vi "Acquisition.vi"(7 "Name(\"\" to use uuid)":string="Acquisition") -> ()   [LabVIEW 2017, in "Acquisition.lvlib"]
uses:
  Acquisition.lvlib
  _support/Hardware Configuration.ctl
  _support/Signal Type.ctl
  bc6f9ce3-7135-4df3-9fce-67397201bd09.vi
  f3e3012a-dc83-45d7-82c5-490bef76f43f.vi
  e2413101-be31-4c43-921b-7e7496268bc5.vi
  07cbb487-6694-43fd-ac53-f2be3466fcff.vi
  fecb174d-6823-407c-a974-ffebb4610b14.vi
  0bf643a1-791c-4b4c-b91f-da80b9c7e2fb.vi
  041ba748-83ae-40d3-86c4-8e2f4b565384.vi
  <userlib>/_NEVSTOP/Communicable State Machine(CSM)/AdvanceAPI/CSM - Revert Arguments-Safe String.vi
  <userlib>/_NEVSTOP/Communicable State Machine(CSM)/_Shared/Trim Single-line Text.vi
  <userlib>/_NEVSTOP/Communicable State Machine(CSM)/AdvanceAPI/CSM - Make String Arguments Safe.vi
  <userlib>/_NEVSTOP/Communicable State Machine(CSM)/AdvanceAPI/CSM - Break Down Multiple States String.vi
  <userlib>/_NEVSTOP/Communicable State Machine(CSM)/AdvanceAPI/CSM - Compact Multiple States.vi
  f3e3012a-dc83-45d7-82c5-490bef76f43f.vi/99de0c97-112a-4c86-9094-c187659127e1.vi
  <userlib>/_NEVSTOP/Communicable State Machine(CSM)/Utility/Build Error Cluster.vi
  0bf643a1-791c-4b4c-b91f-da80b9c7e2fb.vi/99de0c97-112a-4c86-9094-c187659127e1.vi
  <userlib>/_NEVSTOP/Communicable State Machine(CSM)/AdvanceAPI/CSM - Keywords.vi
  <vilib>/Utility/Data Type/Get Type Information.vi
  <userlib>/_NEVSTOP/Communicable State Machine(CSM)/addons/API-String-Arugments-Support/_Support/Data To SingleElementsArray_csm.vi
  <userlib>/_NEVSTOP/Communicable State Machine(CSM)/addons/API-String-Arugments-Support/_Support/Data To API String Arguments.vi
  <userlib>/_NEVSTOP/Communicable State Machine(CSM)/addons/INI-Static-Variable-Support/_Support/Parse Used Session and Name.vi
  <userlib>/_NEVSTOP/Communicable State Machine(CSM)/addons/INI-Static-Variable-Support/_Support/INI-FGV(lvlibp).vi
  <userlib>/_NEVSTOP/Communicable State Machine(CSM)/addons/INI-Static-Variable-Support/_Support/Populate String with INI Variable.vi
  <userlib>/_NEVSTOP/Communicable State Machine(CSM)/addons/API-String-Arugments-Support/_Support/Convert API String Arguments to Data(variant).vi
  <userlib>/_NEVSTOP/Communicable State Machine(CSM)/addons/API-String-Arugments-Support/_Support/SingleElementsArray To Data_csm.vi
  <userlib>/_NEVSTOP/Communicable State Machine(CSM)/addons/API-String-Arugments-Support/_Support/Query Data as API String Arguments(variant).vi
  <userlib>/_NEVSTOP/Communicable State Machine(CSM)/addons/MassData-Parameter/_support/FGV-MassData(lvlibp).vi
  <userlib>/_NEVSTOP/Communicable State Machine(CSM)/_Polymophic/Add State(s) to Queue By BOOL(Element).vi
  <userlib>/_NEVSTOP/Communicable State Machine(CSM)/_Polymophic/CSM - Filter Duplicated Lines.vi
  <userlib>/_NEVSTOP/Communicable State Machine(CSM)/_Polymophic/CSM - Replace Marks in Messages.vi
  <userlib>/_NEVSTOP/Communicable State Machine(CSM)/Communicable State Machine.lvlib
  <userlib>/_NEVSTOP/Communicable State Machine(CSM)/addons/Loop-Support/CSM Loop Support.lvlib
  <userlib>/_NEVSTOP/Communicable State Machine(CSM)/_Shared/CSM Shared.lvlib
panel:
  in  "Signal Type":enum16{"Sine Wave", "Square with Noise"}(ring)
  in  "Cancel Button":bool
  in  "OK Button":bool
  out "Error Occurred":errorcluster
  out "State History":string
  # "Configure The Simulated Waveform Type"
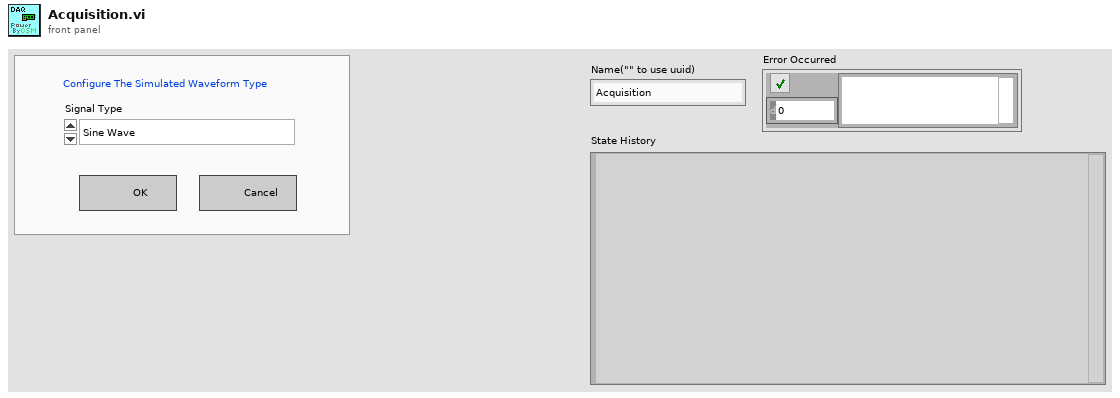
[diagram p1: front panel]
types:
  T1 = enum32{"Invalid", "Default", "Floating", "Floating/Auto-Hide", "Modal"}
  T2 = typedef "Acquisition.lvlib/Hardware Configuration.ctl" = cluster{"Resource":string, "SignalType":T3}
  T3 = typedef "Acquisition.lvlib/Signal Type.ctl" = enum16{"Sine Wave", "Square with Noise"}
  T4 = enum32{"Invalid", "Standard", "Closed", "Hidden", "Minimized", "Maximized"}
  T5 = enum32{"invalid app kind", "Development System", "Run Time System", "Student Edition", "Embedded LabVIEW", "Evaluation", "Custom"}
  T6 = typedef "Communicable State Machine.lvlib/_CSM_Response Source Message.ctl" = cluster{"‘State":string, "’Arguments":string, "’Error":errorcluster}
  T7 = cluster{"Current VI Reference":refnum<vi>, "Close Panel on Exit?":bool}
  T8 = cluster{"Core":cluster{"Current VI Reference":refnum<vi>, "Close Panel on Exit?":bool}, "Configuration":T2, "State":enum16{"Idle", "Acquiring"}, "SamplePeroid(ms)":u32}
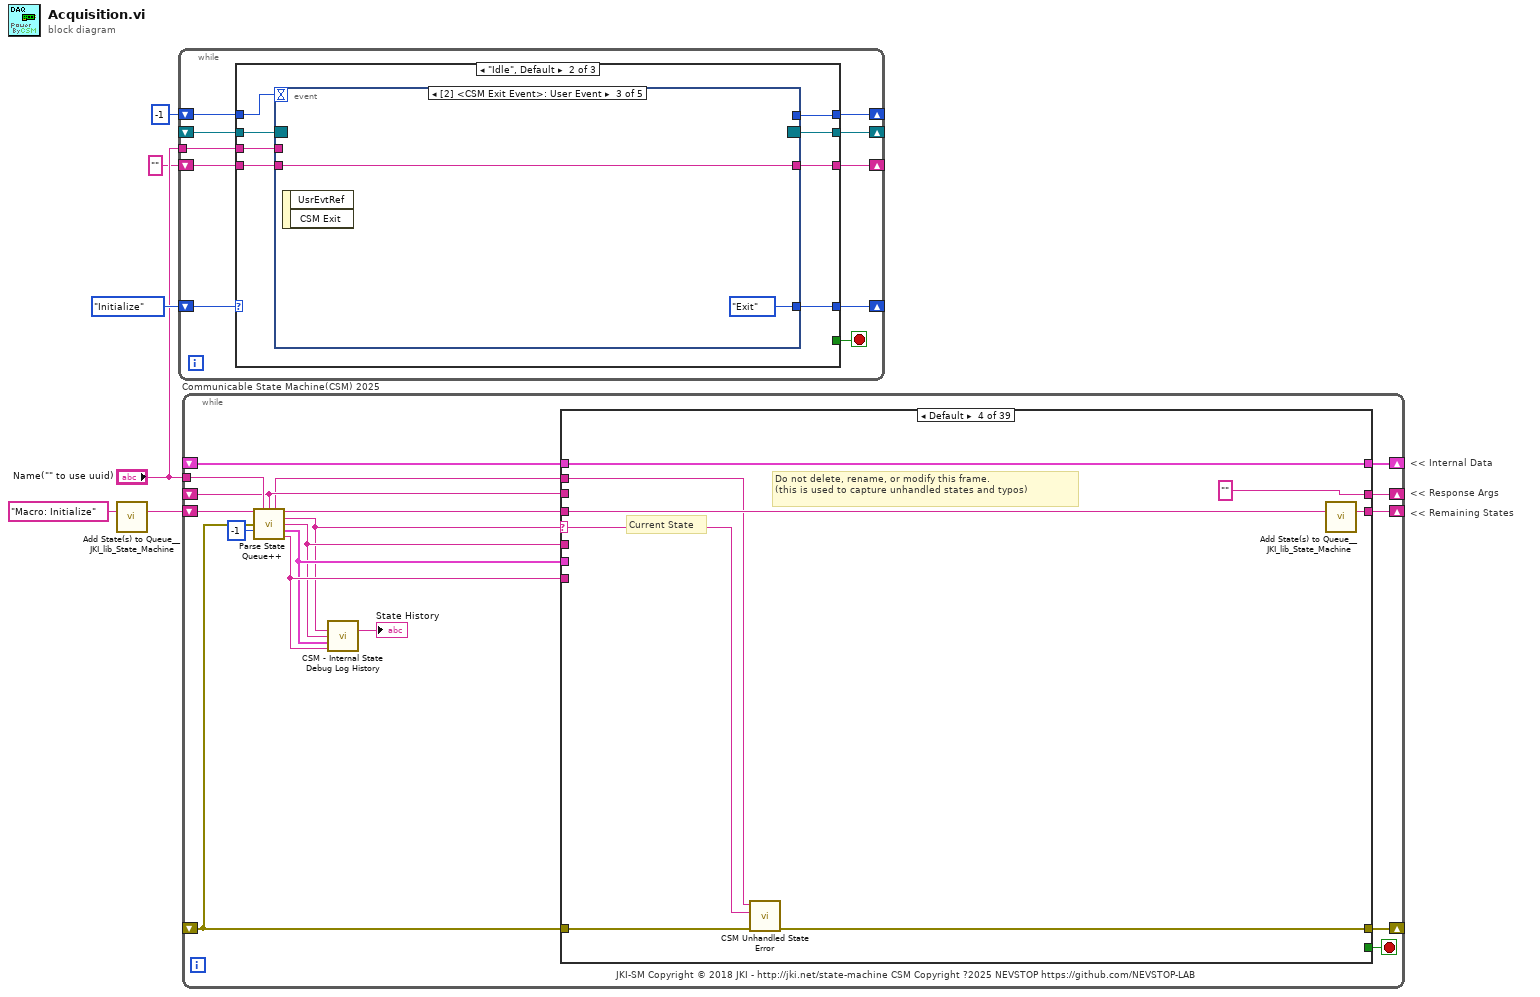
[diagram p0: block diagram]
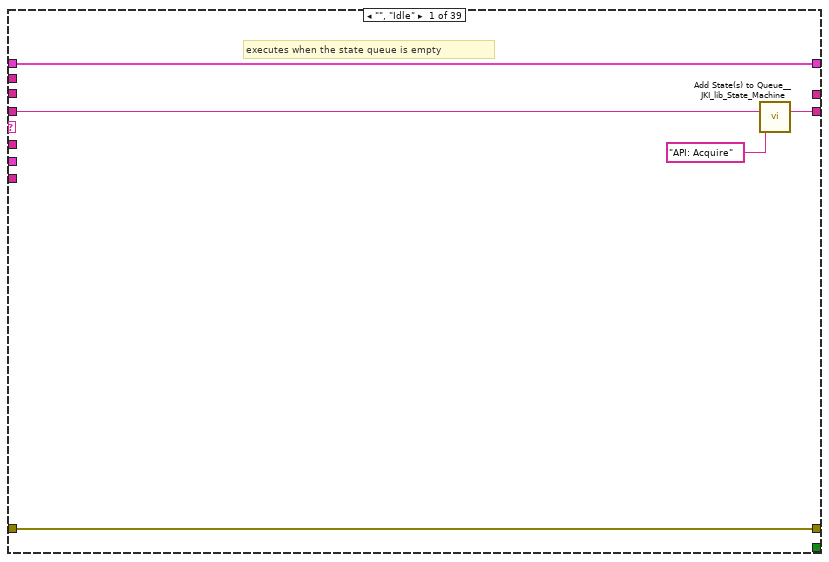
[diagram p2: hidden frame]
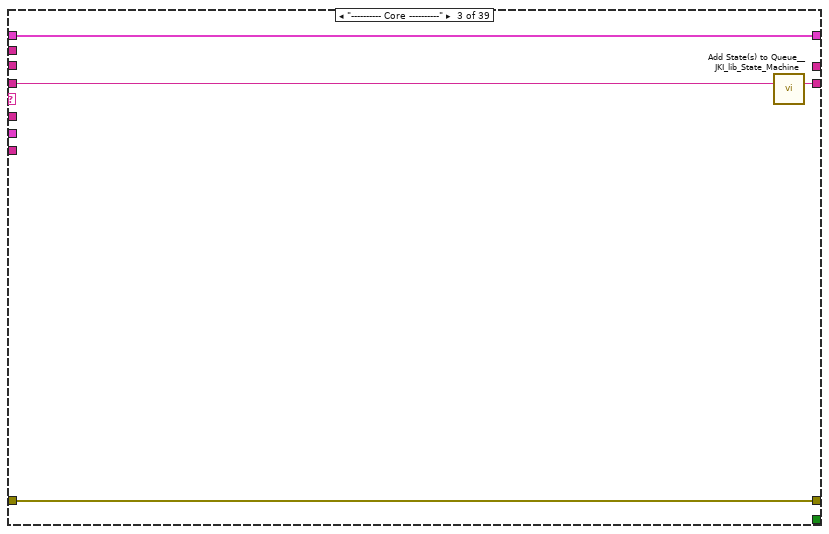
[diagram p4: hidden frame]
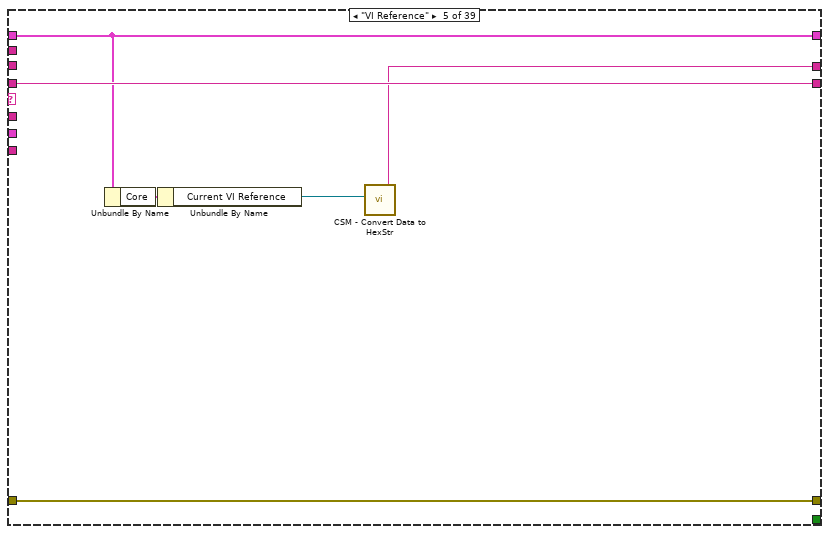
[diagram p5: hidden frame]
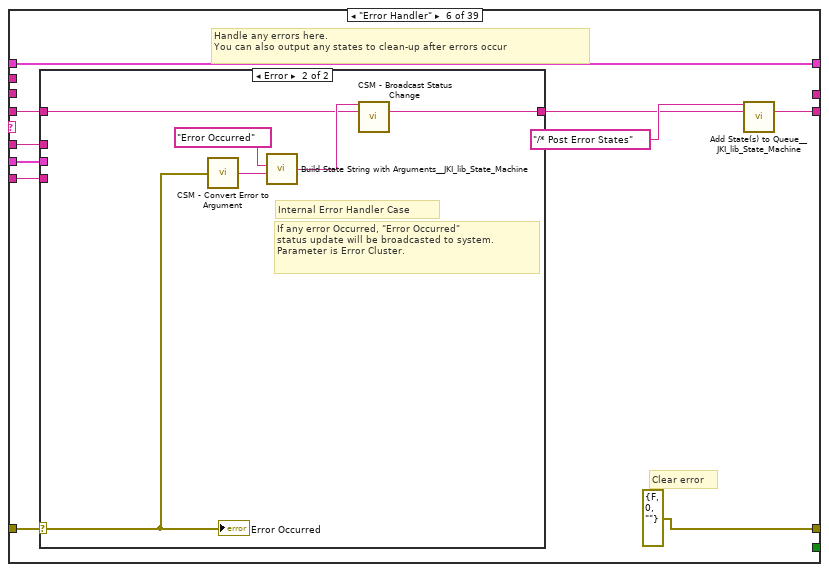
[diagram p6: hidden frame]
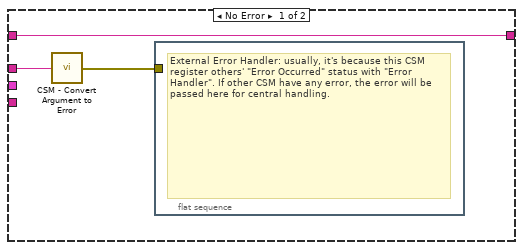
[diagram p7: hidden frame]
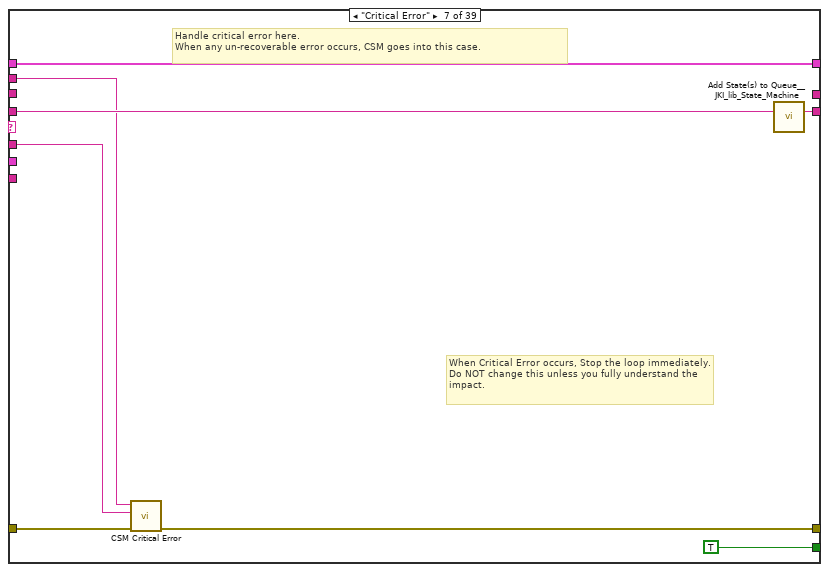
[diagram p8: hidden frame]
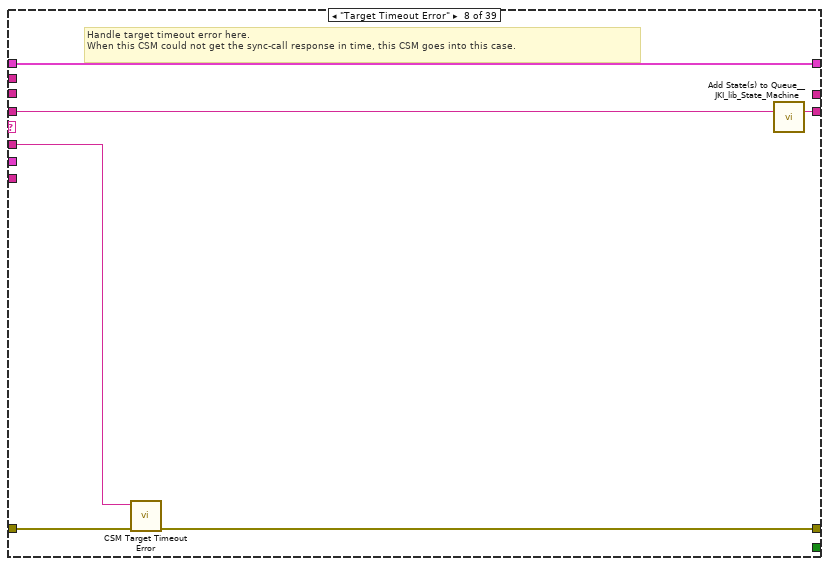
[diagram p9: hidden frame]
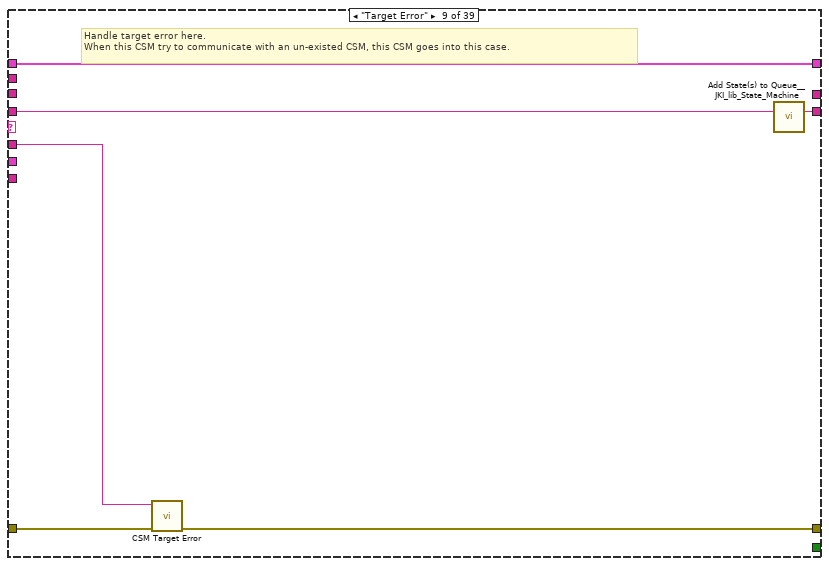
[diagram p10: hidden frame]
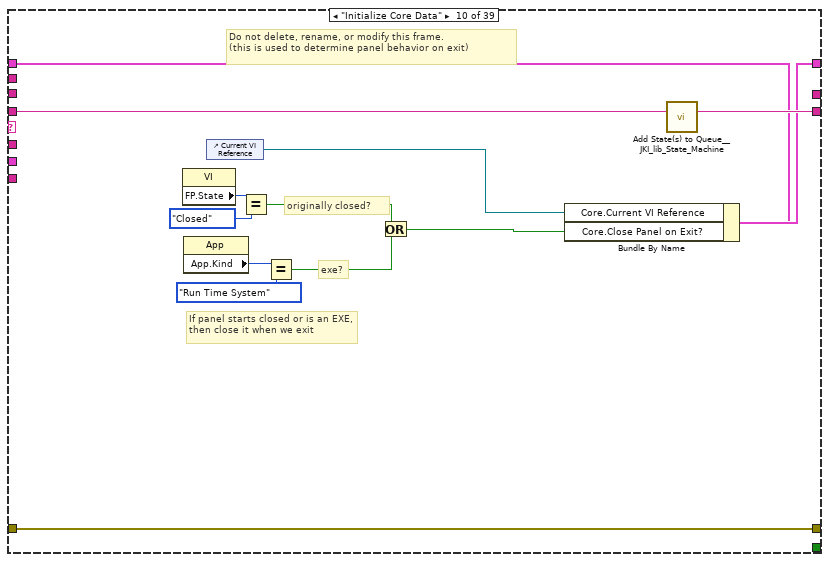
[diagram p11: hidden frame]
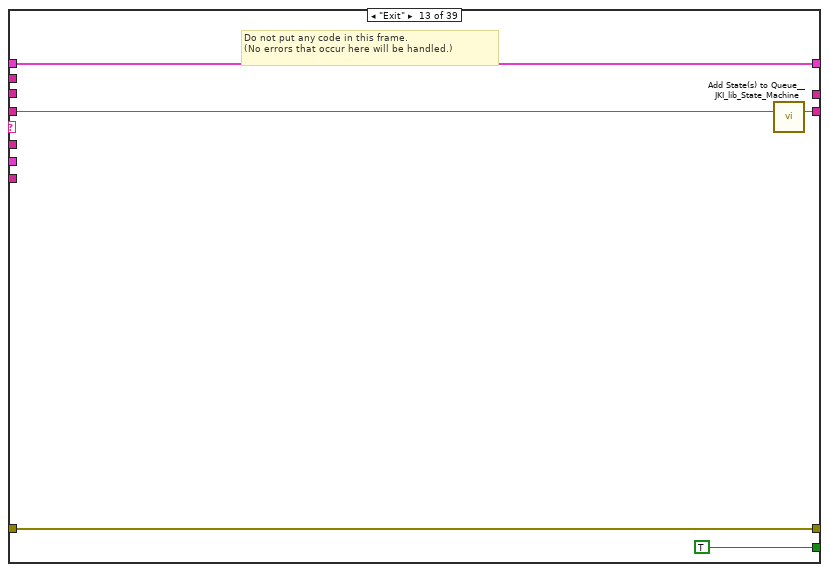
[diagram p14: hidden frame]
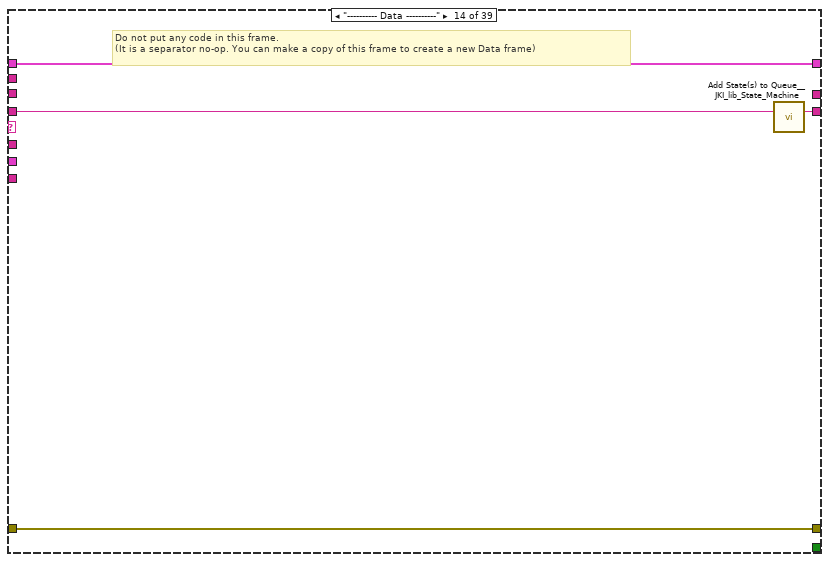
[diagram p15: hidden frame]
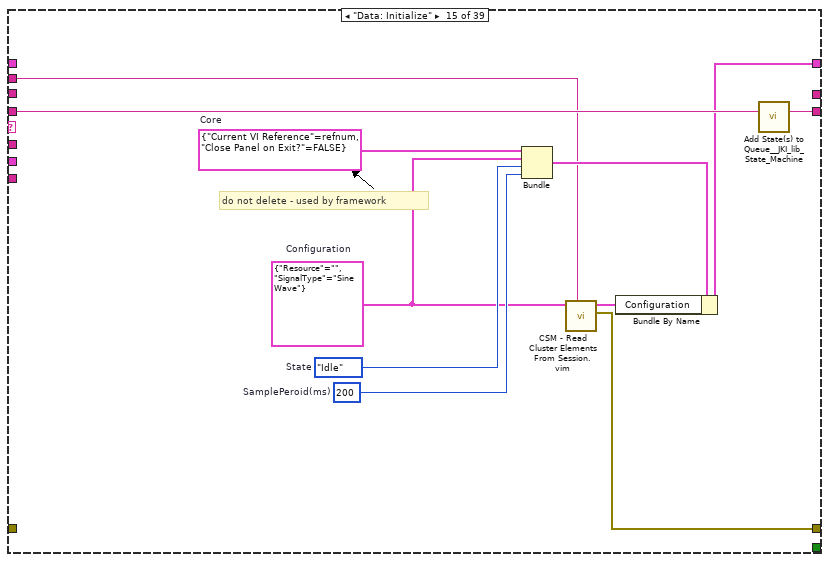
[diagram p16: hidden frame]
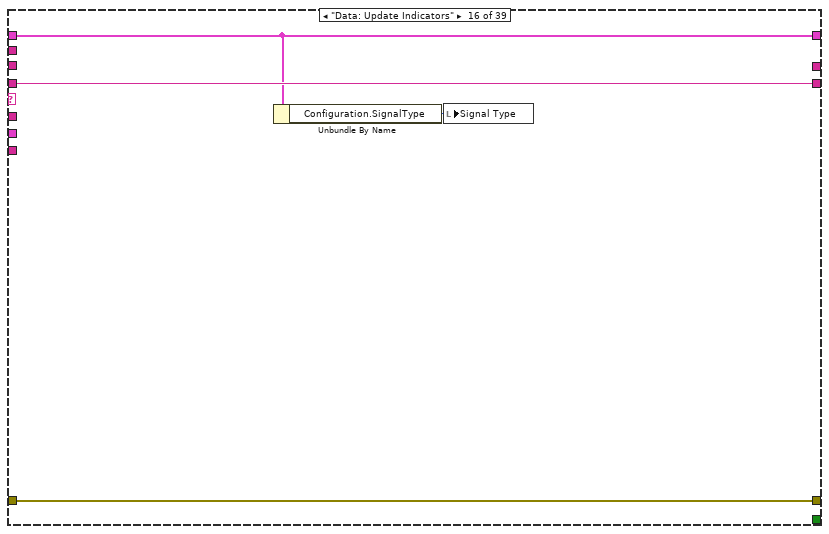
[diagram p17: hidden frame]
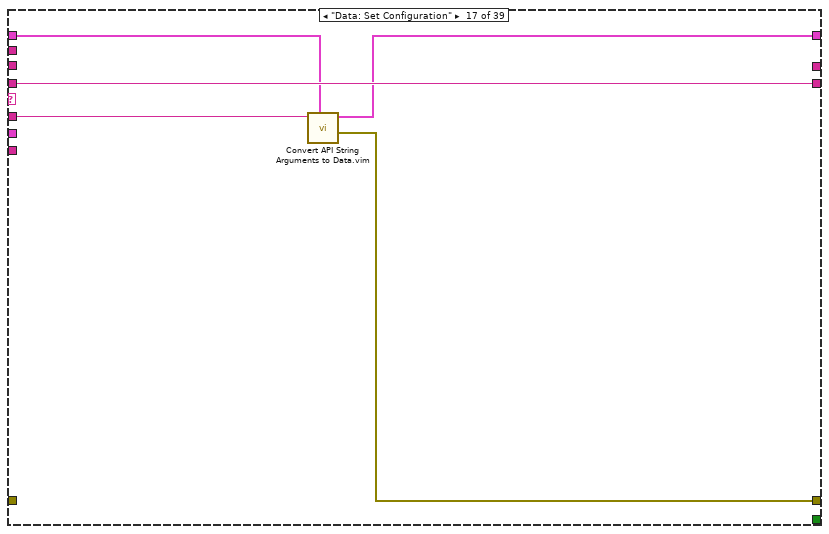
[diagram p18: hidden frame]
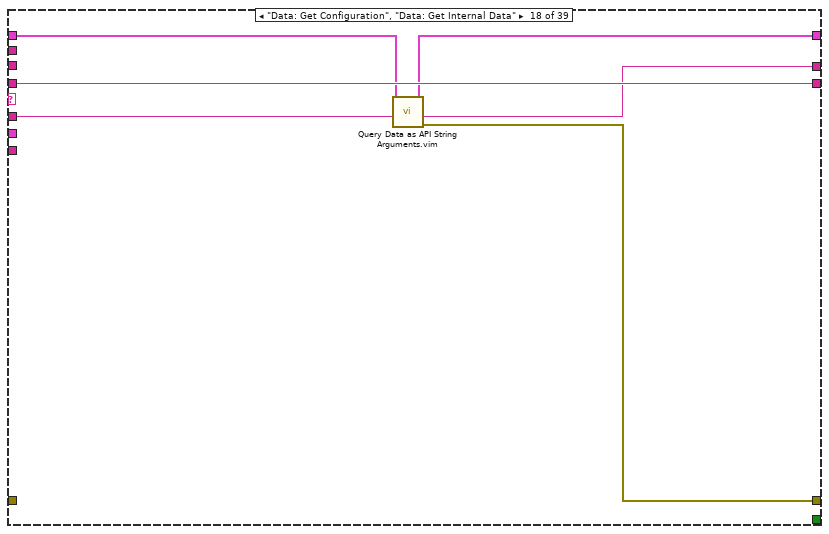
[diagram p19: hidden frame]
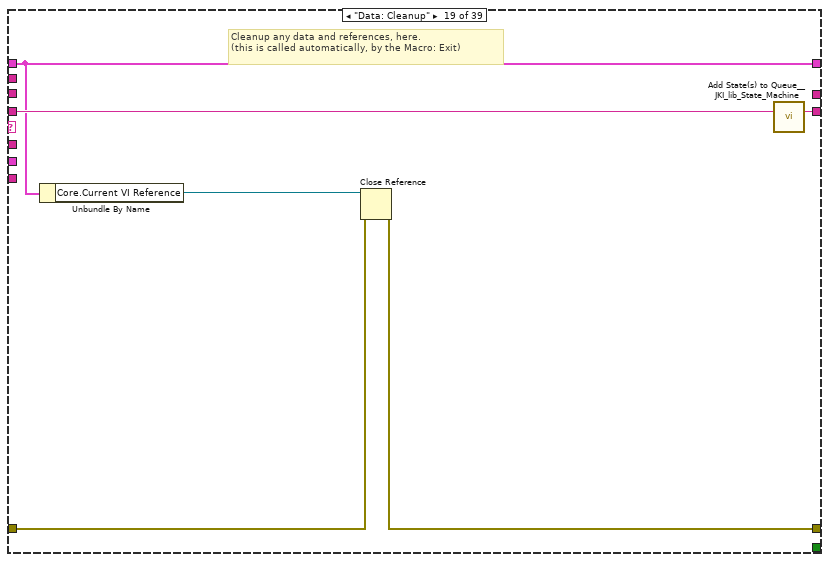
[diagram p20: hidden frame]
diagram:
  # "<< Internal Data"
  # "<< Response Args"
  # "<< Remaining States"
  n1 = call <vilib>:"Add State(s) to Queue__JKI_lib_State_Machine.vi"("State(s) in (\"\")"="Macro: Initialize") -> ("States Out"=w5:string)  [unwired: 14 in]
  n2 = while {
    shift-right: [w12] -> _
    shift-left: enum16{"Idle", "Initialize", "Exit"}."Initialize" -> [w16]
    tunnel: "Name(\"\" to use uuid)" -> [w15]
    shift-right: [w14] -> _
    shift-left: _ -> [w13]
    shift-right: [w9] -> _
    shift-left: "" -> [w10]
    shift-right: [w7] -> _
    shift-left: -1 -> [w8]
    stop <- w11 stop-if-true
    n3 = case shown="\"Idle\", Default" w16 {
      tunnel: w15 -> [w25 w29 _]
      tunnel: [w22 w34 _] -> w14
      tunnel: w13 -> [_ w33 w62]
      tunnel: [enum16{"Idle", "Initialize", "Exit"}."Idle" w32 _] -> w12
      tunnel: [_ _ TRUE] -> w11
      tunnel: w10 -> [w19 w31 w59]
      tunnel: [w19 w30 w59] -> w9
      tunnel: w8 -> [w18 w27 w58]
      tunnel: [w18 w28 w58] -> w7
      frame "Initialize" {
        n4 = call <userlib>:"CSM - Wait for Module to Be Alive.vi"("CSM Name"=w25) -> ("CSM Name (Dup)"=w20:string, "error out"=w26:errorcluster)  [unwired: 12 in, 1 out]
        n5 = call <userlib>:"CSM - Module Exit Event.vi"("Error In"=w26, "Name (\"\" to Use UUID) In"=w20) -> ("error out"=w24:errorcluster, "CSM Exit Event"=w23:refnum<user-event>)  [unwired: 7 in, 1 out]
        n6 = register-events(error in=w24, w23) -> (reference out=w22:refnum<event-registration>)  [unwired: 1 in, 1 out]
        n7 = property class="VI"("FP.Behavior"=T1."Default" ("Front Panel Window:Behavior")) -> ()  [unwired: 2 in, 2 out]
      }
      frame "Idle", Default {
        n8 = event shown="[2] <CSM Exit Event>: User Event" {
          selector: w33 -> [_ _ _ _ _]
          dyn-events: [_ _ _ _ _] -> w34
          timeout: w27 -> [_ _ _ _ _]
          tunnel: [_ _ enum16{"Idle", "Initialize", "Exit"}."Exit" _ _] -> w32
          tunnel: w31 -> [w38 w42 w44 w53 w56]
          tunnel: [w39 w41 w44 w52 w55] -> w30
          tunnel: w29 -> [w36 _ _ _ _]
          tunnel: [-1 _ _ _ _] -> w28
          event Timeout {
            n9 = event-data() -> ()  [unwired: 1 in, 3 out]
            n10 = call-poly <userlib>:"CSM - Filter JKISM String Queue.vi"("States In"=w38) -> ("States Out"=w35:string)  [unwired: 14 in]
            n11 = call <userlib>:"CSM - Forward UI Operations to CSM.vi"("Name (\"\" to Use UUID)"=w36, "State(s) In (\"\")"=w35) -> ("States Out"=w39:string)  [unwired: 8 in, 1 out]
          }
          event Panel Close? {
            n12 = event-data() -> ()  [unwired: 1 in, 2 out]
            n13 = call <vilib>:"Add State(s) to Queue__JKI_lib_State_Machine.vi"("State(s) in Front (\"\")"="Do: Hide FP and Exit When stand-alone" ("State(s) in Front (\"\")"), "State(s) in (\"\")"=w42) -> ("States Out"=w41:string)  [unwired: 13 in]
            n14 = event-data("Discard?"=TRUE) -> ()  [unwired: 1 in, 1 out]
          }
          event User Event {
            n15 = event-data() -> ()  [unwired: 1 in, 2 out]
          }
          event "OK Button": Value Change {
            n16 = event-data() -> ()  [unwired: 1 in, 1 out]
            n17 = Bundle By Name(cluster=T2 {"Resource"="", "SignalType"=enum."Sine Wave"} ("Hardware Config"), "SignalType"="Signal Type") -> (w48:T2)
            n18 = call "Convert Data To API String Arguments.vim"("Data"=w48) -> ("API String"=w47:string)  [unwired: 7 in, 1 out]
            n19 = call-poly <userlib>:"Build Message with Arguments++.vi"("States With Replace Token"="API: Update Settings >> <param>\nData: Update Indicators\nDo: Hide FP and Exit When stand-alone" ("State"), "<param>"=w47) -> ("States"=w46:string)  [unwired: 13 in]
            n20 = call <vilib>:"Add State(s) to Queue__JKI_lib_State_Machine.vi"("State(s) in (\"\")"=w53, "State(s) at Back (\"\")"=w46) -> ("States Out"=w52:string)  [unwired: 13 in]
          }
          event "Cancel Button": Value Change {
            n21 = event-data() -> ()  [unwired: 1 in, 1 out]
            n22 = call <vilib>:"Add State(s) to Queue__JKI_lib_State_Machine.vi"("State(s) in Front (\"\")"="Do: Hide FP and Exit When stand-alone" ("State(s) in Front (\"\")"), "State(s) in (\"\")"=w56) -> ("States Out"=w55:string)  [unwired: 13 in]
          }
        }
      }
      frame "Exit" {
        n23 = Unregister For Events(event registration refnum=w62) -> (error out=w61:errorcluster)  [unwired: 1 in]
        n24 = call <vilib>:"Clear Errors.vi"("error in (no error)"=w61) -> ()  [unwired: 5 in, 2 out]
        n25 = property class="VI"("FP.Behavior"=T1."Default" ("Front Panel Window:Behavior")) -> ()  [unwired: 2 in, 2 out]
      }
    }
  }
  n26 = while "Communicable State Machine(CSM) 2025" {
    shift-right: [w75] -> _
    shift-left: _ -> [w65]
    shift-right: [w78] -> _
    shift-left: _ -> [w74]
    shift-right: [w77] -> _
    shift-left: w5 -> [w79]
    tunnel: "Name(\"\" to use uuid)" -> [w72]
    shift-right: [w73] -> _
    shift-left: _ -> [w67]
    stop <- w76 stop-if-true
    # "JKI-SM Copyright © 2018 JKI - http://jki.net/state-machine CSM Copyright ?2025 NEVSTOP https://github.com/NEVSTOP-LAB"
    n27 = call <userlib>:"Parse State Queue++.vi"("State Queue"=w79, "Name (\"\" to Use UUID)"=w72, "Response Arguments"=w67, "Previous Error"=w74, "Dequeue (1 ms)"=-1 ("Dequeue Timeout(1ms)")) -> ("Name Used"=w66:string, "Remaining States"=w80:string, "Current State"=w68:string, "Arguments"=w69:string, "Additional Information"=w70:T6, "Source CSM"=w71:string)  [unwired: 5 in]
    n28 = call <userlib>:"CSM - Internal State Debug Log History.vi"("State"=w68, "Arguments (\"\")"=w69, ">> Response Source Message >>"=w70, "Source (\"\")"=w71) -> ("Debug Log"=→"State History":string)  [unwired: 11 in]
    n29 = case shown="Default" w68 {
      selector: w68 -> [_ _ _ w94 _ _ _ _ _ _ _ _ _ _ _ _ _ _ _ _ _ _ _ _ _ _ _ _ _ _ _ _ _ _ w316 _ _ _ _]
      tunnel: w80 -> [w82 w87 w92 w99 w105 w110 w132 w138 w144 w158 w160 w163 w169 w173 w184 w187 w193 w199 w205 w209 w214 w219 w221 w225 w238 w251 w262 w269 w275 w280 w285 w308 w310 w313 w320 w323 w327 w334 w401]
      tunnel: w69 -> [_ _ _ _ _ w109 w128 w135 w141 _ _ _ _ _ _ _ w191 w196 _ _ _ _ _ _ _ w247 _ _ _ _ _ _ _ _ w315 _ _ w331 _]
      tunnel: w65 -> [w84 w86 w89 w97 w104 w115 w130 w136 w142 w151 w159 w162 w167 w170 _ w185 w192 w198 w200 w206 w211 w216 w220 w228 w234 w249 w261 w267 w272 w279 w287 w305 w309 w312 w318 w324 w326 w333 w410]
      tunnel: [w85 w88 w90 w95 w106 errorcluster {"status"=FALSE, "code"=0, "source"=""} ("error out") w126 w134 w140 w155 w161 w164 w166 w171 w174 w188 w189 w194 w201 w207 w212 w217 w222 w226 w236 w243 w263 w264 w270 w281 w289 w306 w311 w314 w321 w325 w328 w330 w409] -> w78
      tunnel: w74 -> [w85 w88 w90 w100 w106 w113 w133 w139 w145 w155 w161 w164 w166 w171 _ w188 _ _ w202 w207 w212 w217 w222 w226 w236 _ w263 _ _ w281 w290 _ w311 w314 w321 w325 w328 w332 w409]
      tunnel: [w83 w87 w91 w98 w105 w111 w131 w137 w143 w157 w160 w163 w168 w172 w183 w187 w193 w199 w204 w208 w213 w218 w221 w224 w237 w251 w262 w269 w275 w280 w286 w308 w310 w313 w319 w322 w327 w334 w402] -> w77
      tunnel: [_ _ _ _ _ _ TRUE _ _ _ _ _ TRUE _ _ _ _ _ _ _ _ _ _ _ _ _ _ _ _ _ _ _ _ _ _ _ _ _ _] -> w76
      tunnel: [w84 w86 w89 w97 w104 w115 w130 w136 w142 w156 w159 w162 w167 w170 w176 w185 w190 w197 w200 w206 w211 w216 w220 w227 w234 w250 w261 w265 w271 w278 w288 w304 w309 w312 w318 w324 w326 w333 w410] -> w75
      tunnel: w71 -> [_ _ _ _ _ w108 _ _ _ _ _ _ _ _ _ _ _ _ _ _ _ _ _ _ _ _ _ _ _ _ _ _ _ _ _ _ _ _ _]
      tunnel: w70 -> [_ _ _ _ _ w107 _ _ _ _ _ _ _ _ _ _ _ _ _ _ _ _ _ _ _ _ _ _ _ _ _ _ _ _ _ _ _ _ _]
      tunnel: [_ _ _ "" w101 _ _ _ _ _ _ _ _ _ _ _ _ w195 _ _ _ _ _ _ _ _ _ _ _ _ w283 _ _ _ _ _ _ _ _] -> w73
      tunnel: w66 -> [_ _ _ w93 _ _ w127 _ _ _ _ _ _ _ w178 _ _ _ _ _ _ _ _ _ _ w242 _ _ _ _ _ _ _ _ _ _ _ _ _]
      tunnel: w67 -> [_ _ _ _ _ _ _ _ _ _ _ _ _ _ _ _ _ _ _ _ _ _ _ _ _ _ _ _ _ _ _ _ _ _ _ _ _ _ _]
      frame "", "Idle" {
        # "executes when the state queue is empty"
        n30 = call <vilib>:"Add State(s) to Queue__JKI_lib_State_Machine.vi"("State(s) in (\"\")"=w82, "State(s) at Back (\"\")"="API: Acquire" ("State(s) in Front (\"\")")) -> ("States Out"=w83:string)  [unwired: 13 in]
      }
      frame "CSM Documentation" {
        # "CSM Documentation"
        # "State Syntax:\nStateCategory: State >> Argument -@ CSMName\nStateCategory: State >> Argument -> CSMName\n\nLine Terminator: Line feed"
        # "Commenting:\nTo add a comment use \"//\" or \"#\" and all text to the right will be ignored\nCommenting Example:\nUI: Initialize // This initializes the UI\n// Another comment line"
        # "Example:\nUI: Help >> About -@Main\nUI: Help >> About ->Main\n\nWhere \"UI\" is the state category\nWhere \"Help\" is the state\nWhere \"About\" is the argument\nWhere \"Main\" is the Name of CSM,which actually run the \"UI: Help >> About\"\n\n    \"-@\" stands for sync state. Current CSM will wait until the state is finished. \n            - if \"Main\" named CSM does not exist, \"Target Error\" will occur.\n            - if \"Main\" named CSM is in another sync remote state, \"Target Busy Error\" will occur.\n            - if \"Main\" named CSM could not finish the state in time, \"Target Timeout Error\" will occur.\n            - if everything is right. \"Response\" will occur with Argument back from \"Main\" named CSM. \n\n    \"->\" stands for async state. Current CSM will post the state and continue to next state in next iteration.\n            - if \"Main\" named CSM does not exist, \"Target Error\" will occur.\n            - if everything is right. \"Async Message Posted\" will occur.\n            - After State is finished. Caller will receive a \"Async Response\" state from callee.\n\nWhen duplicated name is used for multiple CSM module or some framework problem happens, \"Critical Error\" will occur."
      }
      frame "---------- Core ----------" {
        n31 = call <vilib>:"Add State(s) to Queue__JKI_lib_State_Machine.vi"("State(s) in (\"\")"=w92) -> ("States Out"=w91:string)  [unwired: 14 in]
      }
      frame Default {
        # "Current State"
        # "Do not delete, rename, or modify this frame.\n(this is used to capture unhandled states and typos)"
        n32 = call <userlib>:"CSM Unhandled State Error.vi"("error in (no error)"=w100, "Undefined State"=w94, "CSM Name"=w93) -> ("error out"=w95:errorcluster)  [unwired: 8 in]
        n33 = call <vilib>:"Add State(s) to Queue__JKI_lib_State_Machine.vi"("State(s) in (\"\")"=w99) -> ("States Out"=w98:string)  [unwired: 14 in]
      }
      frame "VI Reference" {
        n34 = Unbundle By Name(w104) -> ("Core"=w103:T7)
        n35 = Unbundle By Name(w103) -> ("Current VI Reference"=w102:refnum<vi>)
        n36 = call <userlib>:"CSM - Convert Data to HexStr.vi"("Variant"=w102) -> ("HEX String (0-9,A-F)"=w101:string)  [unwired: 8 in]
      }
      frame "Error Handler" {
        # "Handle any errors here.\nYou can also output any states to clean-up after errors occur"
        # "Clear error"
        n37 = case shown="Error" w113 {
          selector: w113 -> [_ w120]
          tunnel: [w119 w122] -> w112
          tunnel: w110 -> [w119 w121]
          tunnel: w109 -> [w118 _]
          tunnel: w108 -> [_ _]
          tunnel: w107 -> [_ _]
          frame No Error {
            n38 = call <userlib>:"CSM - Convert Argument to Error.vi"("Argument"=w118) -> ("Error"=w117:errorcluster)  [unwired: 4 in]
            n39 = flat-sequence {
              tunnel: w117 -> [_]
              frame #0 {
                # "External Error Handler: usually, it's because this CSM register others' \"Error Occurred\" status with \"Error Handler\". If other CSM have any error, the error will be passed here for central handling."
              }
            }
          }
          frame Error {
            # "Internal Error Handler Case"
            # "If any error Occurred, \"Error Occurred\" \nstatus update will be broadcasted to system.\nParameter is Error Cluster."
            n40 = call <userlib>:"CSM - Convert Error to Argument.vi"("Error"=w120) -> ("Argument"=w124:string)  [unwired: 4 in]
            n41 = call <vilib>:"Build State String with Arguments__JKI_lib_State_Machine.vi"("Arguments (\"\")"=w124, "State"="Error Occurred" ("Status with Arguments")) -> ("State with Arguments"=w123:string)  [unwired: 4 in]
            n42 = call <userlib>:"CSM - Broadcast Status Change.vi"("Status With Arguments"=w123, "State Queue"=w121) -> ("Remaining States"=w122:string)  [unwired: 13 in]
            "Error Occurred" <- w120
          }
        }
        n43 = call <vilib>:"Add State(s) to Queue__JKI_lib_State_Machine.vi"("State(s) in Front (\"\")"="/* Post Error States", "State(s) in (\"\")"=w112) -> ("States Out"=w111:string)  [unwired: 13 in]
      }
      frame "Critical Error" {
        # "Handle critical error here.\nWhen any un-recoverable error occurs, CSM goes into this case."
        # "When Critical Error occurs, Stop the loop immediately. Do NOT change this unless you fully understand the impact."
        n44 = call <userlib>:"CSM Critical Error.vi"("error in (no error)"=w133, "Arugments (As Reason)"=w128, "CSM Name"=w127) -> ("error out"=w126:errorcluster)  [unwired: 8 in]
        n45 = call <vilib>:"Add State(s) to Queue__JKI_lib_State_Machine.vi"("State(s) in (\"\")"=w132) -> ("States Out"=w131:string)  [unwired: 14 in]
      }
      frame "Target Timeout Error" {
        # "Handle target timeout error here.\nWhen this CSM could not get the sync-call response in time, this CSM goes into this case."
        n46 = call <userlib>:"CSM Target Timeout Error.vi"("error in (no error)"=w139, "Arguments (As CSM Name)"=w135) -> ("error out"=w134:errorcluster)  [unwired: 9 in]
        n47 = call <vilib>:"Add State(s) to Queue__JKI_lib_State_Machine.vi"("State(s) in (\"\")"=w138) -> ("States Out"=w137:string)  [unwired: 14 in]
      }
      frame "Target Error" {
        # "Handle target error here.\nWhen this CSM try to communicate with an un-existed CSM, this CSM goes into this case."
        n48 = call <userlib>:"CSM Target Error.vi"("error in (no error)"=w145, "Arguments (As CSM Name)"=w141) -> ("error out"=w140:errorcluster)  [unwired: 9 in]
        n49 = call <vilib>:"Add State(s) to Queue__JKI_lib_State_Machine.vi"("State(s) in (\"\")"=w144) -> ("States Out"=w143:string)  [unwired: 14 in]
      }
      frame "Initialize Core Data" {
        # "Do not delete, rename, or modify this frame.\n(this is used to determine panel behavior on exit)"
        # "originally closed?"
        # "exe?"
        # "If panel starts closed or is an EXE, then close it when we exit"
        n50 = property class="VI"() -> ("FP.State"=w148:T4)  [unwired: 2 in, 2 out]
        n51 = property class="App"() -> ("App.Kind"=w154:T5)  [unwired: 2 in, 2 out]
        n52 = control-ref of="Current VI Reference"() -> (w149:refnum<vi>)
        n53 = Equal?(x=w148, y=T4."Closed" ("Front Panel Window:State")) -> (x = y?=w146:bool)
        n54 = Equal?(x=w154, y=T5."Run Time System" ("Application:Kind")) -> (x = y?=w152:bool)
        n55 = Or(x=w146, y=w152) -> (x .or. y?=w150:bool)
        n56 = Bundle By Name(cluster=w151, "Core.Current VI Reference"=w149, "Core.Close Panel on Exit?"=w150) -> (w156:T8)
        n57 = call <vilib>:"Add State(s) to Queue__JKI_lib_State_Machine.vi"("State(s) in (\"\")"=w158) -> ("States Out"=w157:string)  [unwired: 14 in]
      }
      frame "Async Response", "Response" {
      }
      frame "Async Message Posted" {
      }
      frame "Exit" {
        # "Do not put any code in this frame.\n(No errors that occur here will be handled.)"
        n58 = call <vilib>:"Add State(s) to Queue__JKI_lib_State_Machine.vi"("State(s) in (\"\")"=w169) -> ("States Out"=w168:string)  [unwired: 14 in]
      }
      frame "---------- Data ----------" {
        # "Do not put any code in this frame.\n(It is a separator no-op. You can make a copy of this frame to create a new Data frame)"
        n59 = call <vilib>:"Add State(s) to Queue__JKI_lib_State_Machine.vi"("State(s) in (\"\")"=w173) -> ("States Out"=w172:string)  [unwired: 14 in]
      }
      frame "Data: Initialize" {
        w179 = u32 200  # SamplePeroid(ms)
        w180 = enum16{"Idle", "Acquiring"}."Idle"  # State
        w177 = T2 {"Resource"="", "SignalType"=enum."Sine Wave"}  # Configuration
        w181 = T7 {"Current VI Reference"=refnum, "Close Panel on Exit?"=FALSE}  # Core
        # "do not delete - used by framework"
        n60 = Bundle("Core"=w181, "Configuration"=w177, "State"=w180, "SamplePeroid(ms)"=w179) -> (w182:T8)  [unwired: 1 in]
        n61 = call "CSM - Read Cluster Elements From Session.vim"("Section Name (\"\" as Default)"=w178, "Cluster"=w177) -> ("error out"=w174:errorcluster, "Cluster out"=w175:T2)  [unwired: 6 in]
        n62 = Bundle By Name(cluster=w182, "Configuration"=w175) -> (w176:T8)
        n63 = call <vilib>:"Add State(s) to Queue__JKI_lib_State_Machine.vi"("State(s) in (\"\")"=w184) -> ("States Out"=w183:string)  [unwired: 14 in]
      }
      frame "Data: Update Indicators" {
        n64 = Unbundle By Name(w185) -> ("Configuration.SignalType"=w186:T3)
        n65 = local write "Signal Type"(w186) -> ()
      }
      frame "Data: Set Configuration" {
        n66 = call "Convert API String Arguments to Data.vim"("Reference Type"=w192, "API String"=w191) -> ("error out"=w189:errorcluster, "Data"=w190:T8)  [unwired: 6 in]
      }
      frame "Data: Get Configuration", "Data: Get Internal Data" {
        n67 = call "Query Data as API String Arguments.vim"("Name"=w196, "Cluster Data"=w198) -> ("error"=w194:errorcluster, "API String"=w195:string, "Cluster Data (dup)"=w197:T8)  [unwired: 7 in]
      }
      frame "Data: Cleanup" {
        # "Cleanup any data and references, here.\n(this is called automatically, by the Macro: Exit)"
        n68 = Unbundle By Name(w200) -> ("Core.Current VI Reference"=w203:refnum<vi>)
        n69 = Close Reference(reference=w203, error in (no error)=w202) -> (error out=w201:errorcluster)
        n70 = call <vilib>:"Add State(s) to Queue__JKI_lib_State_Machine.vi"("State(s) in (\"\")"=w205) -> ("States Out"=w204:string)  [unwired: 14 in]
      }
      frame "---------- Macro ----------" {
        # "Do not put any code in this frame.\n(It is a separator no-op. You can make a copy of this frame to create a new Macro frame)"
        n71 = call <vilib>:"Add State(s) to Queue__JKI_lib_State_Machine.vi"("State(s) in (\"\")"=w209) -> ("States Out"=w208:string)  [unwired: 14 in]
      }
      frame "Macro: Initialize" {
        # "Initialization Macro\n(This is called once, when the VI starts)"
        n72 = call <vilib>:"Add State(s) to Queue__JKI_lib_State_Machine.vi"("State(s) in Front (\"\")"="Data: Initialize\nInitialize Core Data\nData: Update Indicators", "State(s) in (\"\")"=w214) -> ("States Out"=w213:string)  [unwired: 13 in]
      }
      frame "Macro: Exit" {
        # "Exit Macro\n(This is called once, when the VI exits)"
        n73 = call <vilib>:"Add State(s) to Queue__JKI_lib_State_Machine.vi"("State(s) in Front (\"\")"="Data: Cleanup\nExit", "State(s) in (\"\")"=w219) -> ("States Out"=w218:string)  [unwired: 13 in]
      }
      frame "---------- API ----------" {
        # "Do not put any code in this frame.\n(It is a separator no-op. This category is recommended to use for external API)"
      }
      frame "API: Start" {
        # "#CSM-NOTE\nhttps://github.com/NEVSTOP-LAB/CSM-Continuous-Meausrement-and-Logging/issues/21\n\nUse CSM-Loop Support to define a loop in CSM, which is recommanded."
        # "Copy/Rename this case for your own API"
        n74 = Unbundle By Name(w228) -> ("State"=w229:enum16{"Idle", "Acquiring"})
        n75 = case shown="\"Idle\"" w229 {
          selector: w229 -> [w231 _]
          tunnel: [w231 enum16{"Idle", "Acquiring"}."Acquiring" ("Acquisition State")] -> w230
          tunnel: [_ "DAQ: Initialize \nDAQ: Configure\nDAQ: Start\nDAQ: Acquisite\nContinuous Check >> DAQ: Acquisite -><loop> \nDAQ: Stop\nDAQ: Close " ("State(s) in Front (\"\")")] -> w223
          frame "Acquiring" {
            # "The system is already acquiring. Ignore the \"Start\" message."
          }
          frame "Idle" {
            # "If the system is idle, start the acquisition."
          }
        }
        n76 = call <userlib>:"CSMLS - Define Loop State(s).vi"("Loop States"=w223, "States Queue"=w225) -> ("Remaining States"=w224:string)  [unwired: 13 in]
        n77 = Bundle By Name(cluster=w228, "State"=w230) -> (w227:T8)
      }
      frame "API: Stop" {
        # "Copy/Rename this case for your own API"
        n78 = Unbundle By Name(w234) -> ("State"=w239:enum16{"Idle", "Acquiring"})
        n79 = case shown="\"Acquiring\"" w239 {
          tunnel: ["Break Continuous" ("State(s) in Front (\"\")") _] -> w235
          frame "Acquiring" {
            # "If the system is acquiring, stop the acquisition."
          }
          frame "Idle" {
            # "The system is already idle. Ignore the \"Stop\" message."
          }
        }
        n80 = call <vilib>:"Add State(s) to Queue__JKI_lib_State_Machine.vi"("State(s) in Front (\"\")"=w235, "State(s) in (\"\")"=w238) -> ("States Out"=w237:string)  [unwired: 13 in]
      }
      frame "API: Update Settings" {
        # "#CSM-NOTE\nSync with ini-variable, to make sure the configuration could be stored in CSM INI-Variable configuration file."
        # "#CSM-NOTE\nUse this method to identify the argument type."
        n81 = Unbundle By Name(w249) -> ("Configuration"=w248:T2)
        n82 = call <userlib>:"CSM - Argument Type.vi"("Arguments"=w247) -> ("Argument Type"=w244:string, "Arguments (Dup)"=w245:string)  [unwired: 3 in]
        n83 = case shown="\"HexStr\"" w244 {
          tunnel: w248 -> [w254 w260]
          tunnel: [w253 w259] -> w241
          tunnel: [w252 w258] -> w246
          tunnel: w245 -> [w256 w257]
          frame "HexStr" {
            n84 = call <userlib>:"CSM - Convert HexStr to Data.vi"("HEX String"=w256) -> ("Variant"=w255:variant)  [unwired: 7 in, 1 out]
            n85 = Variant To Data(type=w254, Variant=w255) -> (data=w253:T2, error out=w252:errorcluster)  [unwired: 1 in]
          }
          frame Default {
            n86 = call "Convert API String Arguments to Data.vim"("Reference Type"=w260, "API String"=w257) -> ("error out"=w258:errorcluster, "Data"=w259:T2)  [unwired: 6 in]
          }
        }
        n87 = call "CSM - Write Configuration Variable.vim"("Section Name (\"\" as Default)"=w242, "error in (no error)"=w246, "Configuration"=w241) -> ("error out"=w243:errorcluster)  [unwired: 5 in, 1 out]
        n88 = Bundle By Name(cluster=w249, "Configuration"=w241) -> (w250:T8)
      }
      frame "---------- DAQ ----------" {
      }
      frame "DAQ: Initialize" {
        # "Edit these VIs to configure the acquisition."
        n89 = Unbundle By Name(w267) -> ("Configuration"=w268:T2)
        n90 = call "Initialize Hardware References.vi"("Hardware Resources in"=w268) -> ("error out"=w264:errorcluster, "Hardware Resources out"=w266:T2)  [unwired: 9 in]
        n91 = Bundle By Name(cluster=w267, "Configuration"=w266) -> (w265:T8)
      }
      frame "DAQ: Configure" {
        # "Edit these VIs to configure the acquisition."
        n92 = Unbundle By Name(w272) -> ("Configuration"=w274:T2)
        n93 = call "Configure Hardware.vi"("Hardware Resources in"=w274) -> ("error out"=w270:errorcluster, "Hardware Resources out"=w273:T2)  [unwired: 9 in]
        n94 = Bundle By Name(cluster=w272, "Configuration"=w273) -> (w271:T8)
      }
      frame "DAQ: Start" {
        w277 = u32 200  # SamplePeroid(ms)
        n95 = Bundle By Name(cluster=w279, "SamplePeroid(ms)"=w277, "State"=enum16{"Idle", "Acquiring"}."Acquiring" ("Acquisition State")) -> (w278:T8)
      }
      frame "DAQ: Acquisite" {
        n96 = Unbundle By Name(w287) -> ("State"=w291:enum16{"Idle", "Acquiring"})
        n97 = case shown="\"Acquiring\"" w291 {
          tunnel: [w293 w294] -> w289
          tunnel: w290 -> [w293 w298]
          tunnel: [w292 w299] -> w288
          tunnel: w287 -> [w292 w300]
          tunnel: [_ w296] -> w283
          frame "Idle" {
            # "Ignore \"Acquire\" messages when the acquisition is idle."
          }
          frame "Acquiring" {
            # "Edit these VIs to configure the acquisition."
            # "Acquire more data while in the \"Acquiring\" state."
            n98 = Unbundle By Name(w300) -> ("Configuration.Resource"=w301:string, "Configuration.SignalType"=w302:T3)
            n99 = call "Generate Simulated Data.vi"("error in (no error)"=w298, "Signal Type"=w302) -> ("error out"=w295:errorcluster, "Graph Data"=w297:waveform(dbl)[])  [unwired: 8 in]
            n100 = Bundle By Name(cluster=w300, "Configuration.Resource"=w301, "Configuration.SignalType"=w302) -> (w299:T8)
            n101 = call "CSM - Convert MassData to Argument.vim"("error in (no error)"=w295, "Data"=w297) -> ("error out"=w294:errorcluster, "MassData Argument"=w296:string)  [unwired: 6 in]
          }
        }
        n102 = call <vilib>:"Build State String with Arguments__JKI_lib_State_Machine.vi"("Arguments (\"\")"=w283, "State"="Acquired Waveform" ("Status with Arguments")) -> ("State with Arguments"=w282:string)  [unwired: 4 in]
        n103 = call <userlib>:"CSM - Broadcast Status Change.vi"("Status With Arguments"=w282, "State Queue"=w285) -> ("Remaining States"=w286:string)  [unwired: 13 in]
      }
      frame "DAQ: Stop" {
        n104 = Unbundle By Name(w305) -> ("Configuration"=w307:T2)
        n105 = call "Stop Acquisition.vi"("Hardware Resources in"=w307) -> ("error out"=w306:errorcluster)  [unwired: 10 in]
        n106 = Bundle By Name(cluster=w305, "State"=enum16{"Idle", "Acquiring"}."Idle" ("Acquisition State")) -> (w304:T8)
      }
      frame "DAQ: Close" {
      }
      frame "---------- Control Logic ----------" {
      }
      frame "Continuous Check" {
        n107 = Unbundle By Name(w318) -> ("SamplePeroid(ms)"=w317:u32)
        n108 = Wait (ms)(milliseconds to wait=w317) -> ()  [unwired: 1 out]
        n109 = call <userlib>:"CSMLS - Append Continuous State.vi"("Loop State(s) And Arguments"=w315, "Continous Arguments (\"\")"=w315, "Continous State"=w316, "States Queue"=w320) -> ("Remaining States"=w319:string)  [unwired: 7 in]
      }
      frame "Break Continuous" {
        n110 = call <userlib>:"CSMLS - Remove Loop Tag to Break.vi"("States Queue"=w323) -> ("Remaining States"=w322:string)  [unwired: 10 in]
      }
      frame "---------- DoSth ----------" {
      }
      frame "Do: Front Panel State" {
        n111 = Unbundle By Name(w333) -> ("Core.Current VI Reference"=w329:refnum<vi>)
        n112 = case shown="\"Hidden\", \"Hide\"" w331 {
          tunnel: w332 -> [w340 w355 w366 w379 w392]
          tunnel: [w342 w356 w368 w381 w394] -> w330
          tunnel: w329 -> [w341 w353 w367 w380 w393]
          frame "Open", "Standard", Default {
            w335 = T4."Standard" ("State")
            n113 = property class="VI"(reference=w341, error in=w340) -> (reference out=w338:refnum<vi>, error out=w339:errorcluster, "FP.State"=w337:T4)
            n114 = Not Equal?(x=w337, y=w335) -> (x != y?=w336:bool)
            n115 = case shown="True" w336 {
              tunnel: [w346 w348] -> w342
              tunnel: w339 -> [w345 w348]
              tunnel: w338 -> [w344 _]
              tunnel: w335 -> [w343 _]
              frame True {
                n116 = invoke class="VI" method="FP.Open"(reference=w344, error in=w345, "Activate"=TRUE, "State"=w343) -> (error out=w346:errorcluster)  [unwired: 1 in, 4 out]
              }
              frame False {
              }
            }
          }
          frame "Close", "Closed" {
            n117 = property class="VI"(reference=w353, error in=w355) -> (reference out=w352:refnum<vi>, error out=w354:errorcluster, "FP.State"=w350:T4)
            n118 = Not Equal?(x=w350, y=T4."Closed" ("Front Panel Window:State")) -> (x != y?=w349:bool)
            n119 = case shown="True" w349 {
              tunnel: [w357 w360] -> w356
              tunnel: w354 -> [w357 w359]
              tunnel: w352 -> [_ w358]
              frame False {
              }
              frame True {
                n120 = invoke class="VI" method="FP.Close"(reference=w358, error in=w359) -> (error out=w360:errorcluster)  [unwired: 1 in, 2 out]
              }
            }
          }
          frame "Hidden", "Hide" {
            w361 = T4."Hidden" ("State")
            n121 = property class="VI"(reference=w367, error in=w366) -> (reference out=w364:refnum<vi>, error out=w365:errorcluster, "FP.State"=w363:T4)
            n122 = Not Equal?(x=w363, y=w361) -> (x != y?=w362:bool)
            n123 = case shown="True" w362 {
              tunnel: [w372 w373] -> w368
              tunnel: w365 -> [w371 w373]
              tunnel: w364 -> [w370 _]
              tunnel: w361 -> [w369 _]
              frame True {
                n124 = invoke class="VI" method="FP.Open"(reference=w370, error in=w371, "State"=w369) -> (error out=w372:errorcluster)  [unwired: 2 in, 4 out]
              }
              frame False {
              }
            }
          }
          frame "Minimize", "Minimized" {
            w374 = T4."Minimized" ("State")
            n125 = property class="VI"(reference=w380, error in=w379) -> (reference out=w377:refnum<vi>, error out=w378:errorcluster, "FP.State"=w376:T4)
            n126 = Not Equal?(x=w376, y=w374) -> (x != y?=w375:bool)
            n127 = case shown="True" w375 {
              tunnel: [w385 w386] -> w381
              tunnel: w378 -> [w384 w386]
              tunnel: w377 -> [w383 _]
              tunnel: w374 -> [w382 _]
              frame True {
                n128 = invoke class="VI" method="FP.Open"(reference=w383, error in=w384, "State"=w382) -> (error out=w385:errorcluster)  [unwired: 2 in, 4 out]
              }
              frame False {
              }
            }
          }
          frame "Maximize", "Maximized" {
            w387 = T4."Maximized" ("State")
            n129 = property class="VI"(reference=w393, error in=w392) -> (reference out=w390:refnum<vi>, error out=w391:errorcluster, "FP.State"=w389:T4)
            n130 = Not Equal?(x=w389, y=w387) -> (x != y?=w388:bool)
            n131 = case shown="True" w388 {
              tunnel: [w398 w399] -> w394
              tunnel: w391 -> [w397 w399]
              tunnel: w390 -> [w396 _]
              tunnel: w387 -> [w395 _]
              frame True {
                n132 = invoke class="VI" method="FP.Open"(reference=w396, error in=w397, "State"=w395) -> (error out=w398:errorcluster)  [unwired: 2 in, 4 out]
              }
              frame False {
              }
            }
          }
        }
      }
      frame "Do: Hide FP and Exit When stand-alone" {
        # "#CSM-NOTE\nNo parent"
        n133 = Call Chain() -> (call chain=w406:string[])
        n134 = Array Size(array=w406) -> (size(s)=w405:i32)
        n135 = Equal?(x=1, y=w405) -> (x = y?=w403:bool)
        n136 = call-poly <userlib>:"Add State(s) to Queue By BOOL++.vi"("TRUE (\"\")"="Macro: Exit" ("State(s) at Back (\"\")"), "Condition"=w403, "State Queue (\"\")"="Do: Front Panel State >> Hide" ("State(s) at Back (\"\")")) -> ("Remaining States"=w400:string)  [unwired: 8 in]
        n137 = call <vilib>:"Add State(s) to Queue__JKI_lib_State_Machine.vi"("State(s) in Front (\"\")"=w400, "State(s) in (\"\")"=w401) -> ("States Out"=w402:string)  [unwired: 13 in]
      }
    }
  }
